vi "Display MinMax.vi"(8 "error in (no error)":errorcluster, 10 "Main":refnum<vi>) -> (0 "error out":errorcluster)   [LabVIEW 2025, in "Flow Grind.lvlib" / "No Load Drift.lvclass"]
uses:
  No Load Drift.lvclass
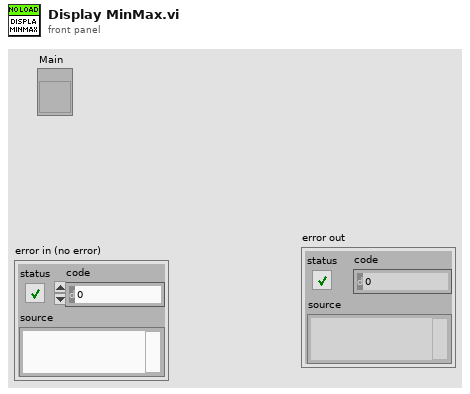
[diagram p1: front panel]
types:
  T1 = typedef "LVAnnotationListTypeDef.ctl" = cluster{"Name":string, "Color":u32, "Style":u8, "Point Style":u8, "Name Visible":bool, "Allow Drag":bool, "Annotation Mode":u32, "Plot":i32, "Index":i32, "Position":cluster{"X":dbl, "Y":dbl}, "X Scale":u32, "Y Scale":u32, "Show Arrow":bool, "Lock Name":bool, "Plot Area":i32, "Label Offset":cluster{"X":dbl, "Y":dbl}}[]
  T2 = cluster{"Name":string, "Color":u32, "Style":u8, "Point Style":u8, "Name Visible":bool, "Allow Drag":bool, "Annotation Mode":u32, "Plot":i32, "Index":i32, "Position":cluster{"X":dbl, "Y":dbl}, "X Scale":u32, "Y Scale":u32, "Show Arrow":bool, "Lock Name":bool, "Plot Area":i32, "Label Offset":cluster{"X":dbl, "Y":dbl}}
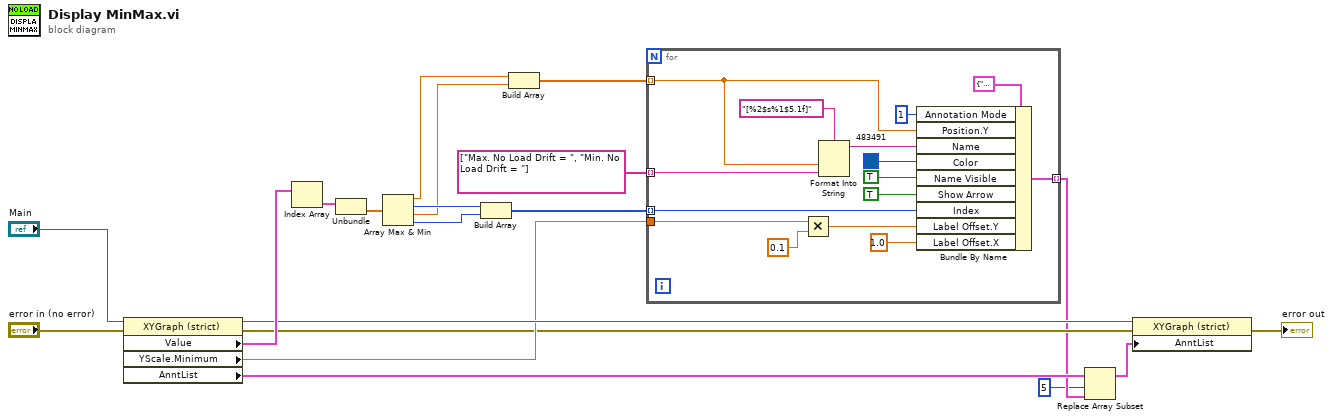
[diagram p0: block diagram]
diagram:
  n1 = property class="XYGraph (strict)"(reference="Main", error in="error in (no error)") -> (reference out=w11:refnum<vi>, error out=w7:errorcluster, "Value"=w15:cluster{dbl[], dbl[]}[], "YScale.Minimum"=w10:dbl, "AnntList"=w6:T1)
  n2 = Index Array(array=w15) -> (element=w14:cluster{dbl[], dbl[]})  [unwired: 1 in]
  n3 = Unbundle(w14) -> (w13:dbl[])  [unwired: 1 out]
  n4 = Array Max & Min(array=w13) -> (max value=w4:dbl, max index (indices)=w18:i32, min value=w3:dbl, min index (indices)=w17:i32)
  n5 = Build Array(w18, w17) -> (w16:i32[])
  n6 = Build Array(w4, w3) -> (w19:dbl[])
  n7 = for {
    tunnel: w19 -> [w21] mode=indexing
    tunnel: string[] ["Max. No Load Drift = ", "Min. No Load Drift = "] -> [w35] mode=indexing
    tunnel: w16 -> [w32] mode=indexing
    tunnel: w10 -> [w28]
    tunnel: [w25] -> w2 mode=indexing
    n8 = Multiply(x=w28, y=0.1) -> (x*y=w26:dbl)
    n9 = Format Into String(format string="[%2$s%1$5.1f]", w21, w35) -> (resulting string=w24:string)  [unwired: 2 in, 1 out]
    n10 = Bundle By Name(cluster=T2 {"Name"="", "Color"=0, "Style"=0, "Point Style"=0, "Name Visible"=FALSE, "Allow Drag"=FALSE, "Annotation Mode"=0, "Plot"=0, "Index"=0, "Position"={"X"=0.0, "Y"=0.0}, "X Scale"=0, "Y Scale"=0, "Show Arrow"=FALSE, "Lock Name"=FALSE, "Plot Area"=0, "Label Offset"={"X"=0.0, "Y"=0.0}}, "Annotation Mode"=u32 1, "Position.Y"=w21, "Name"=w24, "Color"=u32 483491, "Name Visible"=TRUE, "Show Arrow"=TRUE, "Index"=w32, "Label Offset.Y"=w26, "Label Offset.X"=1.0) -> (w25:T2)
  }
  n11 = Replace Array Subset(array=w6, new element=w2, index=5) -> (w5:T1)
  n12 = property class="XYGraph (strict)"(reference=w11, error in=w7, "AnntList"=w5) -> (error out=→"error out":errorcluster)  [unwired: 1 out]
